vi "GetItemType.vi"(11 "Path":path) -> (2 "DNL_Type":T1=enum."Project")   [LabVIEW 2023, in "GettingStartedWindow.lvlib"]
doc: "Based on the file extension, selects a file type. Defaults to VI for unknown extensions."
uses:
  <resource>/modes/FRC/GSW/GettingStartedWindow.lvlib
  <resource>/modes/FRC/GSW/ItemData_Type.ctl
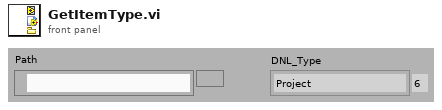
[diagram p1: front panel]
types:
  T1 = typedef "GettingStartedWindow.lvlib/ItemData_Type.ctl" = enum16{"None", "Folder", "New Project", "New VI", "Find", "VI", "Project", "New from template", "RT Project Wizard", "PDA Project Wizard", "Control", "Library", "Class", "XControl", "Runtime menu", "Statechart", "Ladder", "Find LabVIEW Addons", "Instrument Finder", "Example Finder"}
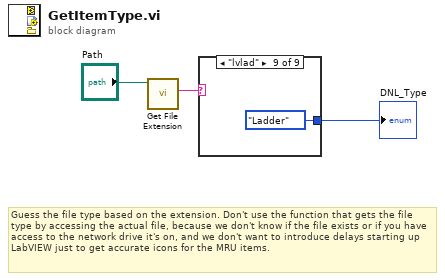
[diagram p0: block diagram]
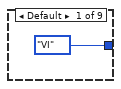
[diagram p2: hidden frame]
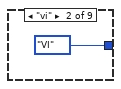
[diagram p3: hidden frame]
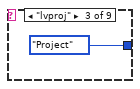
[diagram p4: hidden frame]
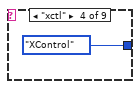
[diagram p5: hidden frame]
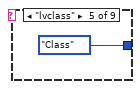
[diagram p6: hidden frame]
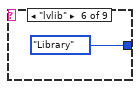
[diagram p7: hidden frame]
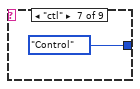
[diagram p8: hidden frame]
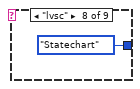
[diagram p9: hidden frame]
diagram:
  # "Guess the file type based on the extension. Don't use the function that gets the file\ntype by accessing the actual file, because we don't know if the file exists or if you have\naccess to the network drive it's on, and we don't want to introduce delays starting up\nLabVIEW just to get accurate icons for the MRU items."
  n1 = call <vilib>:"Get File Extension.vi"("file"="Path") -> ("lowercase file extension"=w1:string)  [unwired: 6 in, 4 out]
  n2 = case shown="\"lvlad\"" w1 {
    tunnel: [ItemData_Type."VI" ("DNL_Type") ItemData_Type."VI" ("DNL_Type") ItemData_Type."Project" ("DNL_Type") ItemData_Type."XControl" ("DNL_Type") ItemData_Type."Class" ("DNL_Type") ItemData_Type."Library" ("DNL_Type") ItemData_Type."Control" ("DNL_Type") ItemData_Type."Statechart" ("DNL_Type") ItemData_Type."Ladder" ("DNL_Type")] -> w3
    frame Default {
    }
    frame "vi" {
    }
    frame "lvproj" {
    }
    frame "xctl" {
    }
    frame "lvclass" {
    }
    frame "lvlib" {
    }
    frame "ctl" {
    }
    frame "lvsc" {
    }
    frame "lvlad" {
    }
  }
  "DNL_Type" <- w3
